vi "Logic.vi"(8 "error in (no error)":errorcluster, 11 "CIFPlugin in":refnum<class "CAN_Reader_CANsub_Plugin.lvclass">) -> (0 "error out":errorcluster, 3 "CIFPlugin out":refnum<class "CAN_Reader_CANsub_Plugin.lvclass">)   [LabVIEW 2021, in "CAN_Reader_CANsub_Plugin.lvclass"]
uses:
  CAN_Reader_CANsub_Plugin.lvclass
  CAN_Reader_CANsub_Plugin.lvclass/CAN_Reader_CANsub_Plugin.ctl
  Common/Typedef/Channels.ctl
  Common/CAN_Reader_CANsub_Common.lvlib
  <vilib>/CIF Foundation/CIF Core/CIFCore/Class/CIFCorePlugin.lvclass
  <vilib>/CIF Foundation/CIF Channels Core/ChannelCommon/typedef/TimeStamps.ctl
  <vilib>/CIF Foundation/CIF Channels Core/ChannelCommon/ChannelCommon.lvlib
  <vilib>/CIF Foundation/CIF Utilities/Time/Time_CIF_U.lvlib
  C:/Program Files/National Instruments/LabVIEW 2021/vi.lib/CIF Foundation/CIF Core/CIFCore/Class/CIFCorePlugin.lvclass
  <vilib>/CIF Foundation/CIF XNET CAN RW/XNET CAN RW.lvclass
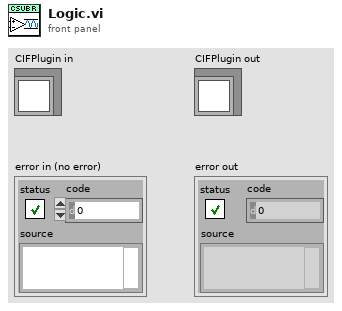
[diagram p1: front panel]
types:
  T1 = typedef "ChannelCommon.lvlib/TimeStamps.ctl" = cluster{"ClockID":u8, "T0":i64, "T_Out":i64}
  T2 = typedef "CAN_Reader_CANsub_Common.lvlib/Channels.ctl" = enum16{"CAN_Frames"}
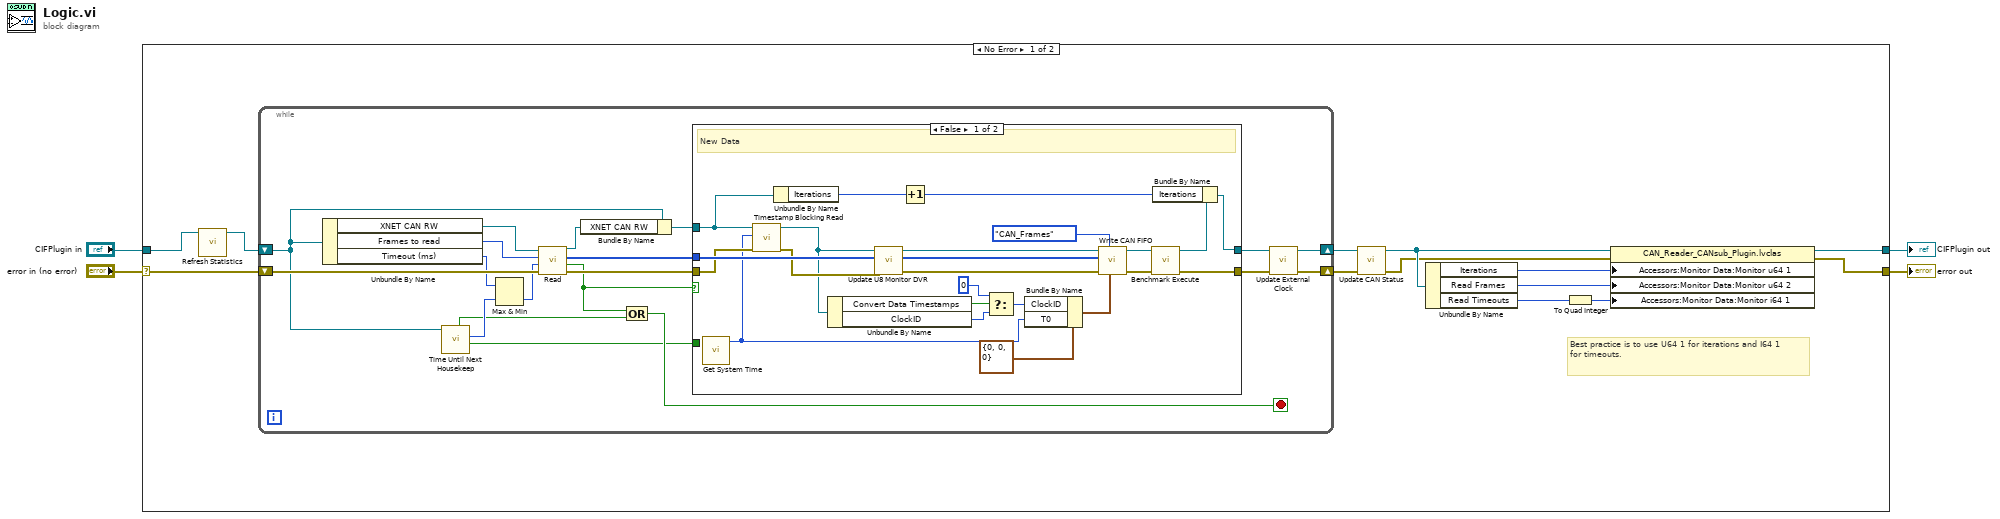
[diagram p0: block diagram]
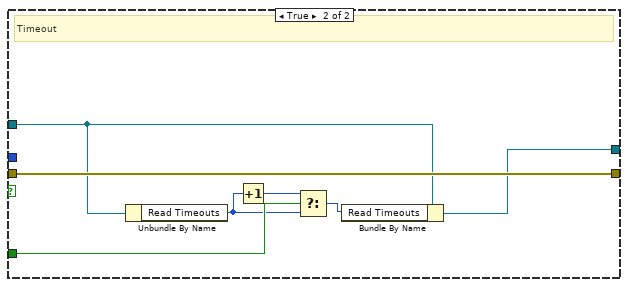
[diagram p2: hidden frame]
diagram:
  n1 = case shown="No Error" "error in (no error)" {
    selector: "error in (no error)" -> [w16 w68]
    tunnel: [w15 w68] -> w2
    tunnel: [w9 w67] -> w1
    tunnel: "CIFPlugin in" -> [w17 w67]
    frame No Error {
      # "Best practice is to use U64 1 for iterations and I64 1 for timeouts."
      n2 = call "Refresh Statistics.vi"("CIFPlugin in"=w17) -> ("CIFPlugin out"=w14:refnum<class "CAN_Reader_CANsub_Plugin.lvclass">)  [unwired: 10 in]
      n3 = while {
        shift-right: [w24] -> w7
        shift-left: w16 -> [w36]
        shift-right: [w25] -> w8
        shift-left: w14 -> [w31]
        stop <- w19 stop-if-true
        n4 = Unbundle By Name(w31) -> ("XNET CAN RW"=w35:refnum<class "XNET CAN RW.lvclass">, "Frames to read"=w34:i32, "Timeout (ms)"=w29:i32)
        n5 = call <vilib>:"Time Until Next Housekeep.vi"("CIFCorePlugin in"=w31) -> ("Timeout Valid"=w18:bool, "Time Until Next Housekeep (ms)"=w30:i32, "Housekeep Now"=w20:bool)  [unwired: 7 in, 1 out]
        n6 = Max & Min(x=w29, y=w30) -> (min(x,y)=w28:i32)  [unwired: 1 out]
        n7 = call-dynamic "Read.vi"("error in (no error)"=w36, "timeout (ms)"=w28, "number to read"=w34, "XNET_CAN_RW in"=w35) -> ("error out"=w22:errorcluster, "Timeout"=w21:bool, "pcap CAN Data"=w33:u8[], "XNET_CAN_RW out"=w32:refnum<class "XNET CAN RW.lvclass">)  [unwired: 3 in, 1 out]
        n8 = Bundle By Name(cluster=w31, "XNET CAN RW"=w32) -> (w23:refnum<class "CAN_Reader_CANsub_Plugin.lvclass">)
        n9 = Compound Arithmetic op=OR(w21, w20) -> (w19:bool)
        n10 = case shown="False" w21 {
          tunnel: w33 -> [w51 _]
          tunnel: w22 -> [w45 w66]
          tunnel: w23 -> [w42 w65]
          tunnel: [w38 w64] -> w27
          tunnel: [w46 w66] -> w26
          tunnel: w18 -> [_ w62]
          frame False {
            # "New Data"
            n11 = call <vilib>:"Get System Time.vi"() -> ("Time (ns)"=w37:i64)  [unwired: 5 in]
            n12 = call <vilib>:"Timestamp Blocking Read.vi"("error in (no error)"=w45, "RX Time"=w37, "CIFCorePlugin in"=w42) -> ("error out"=w44:errorcluster, "CIFCorePlugin out"=w43:refnum<class "CAN_Reader_CANsub_Plugin.lvclass">)  [unwired: 7 in]
            n13 = Unbundle By Name(w42) -> ("Iterations"=w41:u64)
            n14 = Unbundle By Name(w43) -> ("Convert Data Timestamps"=w57:bool, "ClockID"=w56:u8)
            n15 = call "Update U8 Monitor DVR.vi"("error in (no error)"=w44, "pcap CAN Data in"=w51, "CAN_Reader_NIXNET_Plugin in"=w43) -> ("error out"=w49:errorcluster, "pcap CAN Data out"=w50:u8[], "CAN_Reader_NIXNET_Plugin out"=w52:refnum<class "CAN_Reader_CANsub_Plugin.lvclass">)  [unwired: 6 in]
            n16 = Increment(x=w41) -> (x+1=w40:u64)
            n17 = Select(t=u8 0, s=w57, f=w56) -> (s? t:f=w54:u8)
            n18 = Bundle By Name(cluster=T1 {"ClockID"=0, "T0"=0, "T_Out"=0} ("FIFO Timestamps"), "ClockID"=w54, "T0"=w37) -> (w53:T1)
            n19 = call <vilib>:"Write CAN FIFO.vi"("FIFO Timestamps"=w53, "Channel Index"=Channels."CAN_Frames" ("Channels"), "error in (no error)"=w49, "Data"=w50, "CIFCorePlugin in"=w52) -> ("error out"=w47:errorcluster, "CIFCorePlugin out"=w48:refnum<class "CAN_Reader_CANsub_Plugin.lvclass">)  [unwired: 4 in, 1 out]
            n20 = call <vilib>:"Benchmark Execute.vi"("error in (no error)"=w47, "CIFCorePlugin in"=w48) -> ("error out"=w46:errorcluster, "CIFCorePlugin out"=w39:refnum<class "CAN_Reader_CANsub_Plugin.lvclass">)  [unwired: 8 in]
            n21 = Bundle By Name(cluster=w39, "Iterations"=w40) -> (w38:refnum<class "CAN_Reader_CANsub_Plugin.lvclass">)
          }
          frame True {
            # "Timeout"
            n22 = Unbundle By Name(w65) -> ("Read Timeouts"=w60:u64)
            n23 = Increment(x=w60) -> (x+1=w61:u64)
            n24 = Select(t=w61, s=w62, f=w60) -> (s? t:f=w63:u64)
            n25 = Bundle By Name(cluster=w65, "Read Timeouts"=w63) -> (w64:refnum<class "CAN_Reader_CANsub_Plugin.lvclass">)
          }
        }
        n26 = call "Update External Clock.vi"("error in (no error)"=w26, "CAN_Reader_NIXNET"=w27) -> ("error out"=w24:errorcluster, "CAN_Reader_NIXNET"=w25:refnum<class "CAN_Reader_CANsub_Plugin.lvclass">)  [unwired: 8 in]
      }
      n27 = call "Update CAN Status.vi"("error in (no error)"=w7, "CAN_Reader_NIXNET_Plugin"=w8) -> ("error out"=w5:errorcluster, "CAN_Reader_NIXNET_Plugin"=w6:refnum<class "CAN_Reader_CANsub_Plugin.lvclass">)  [unwired: 8 in]
      n28 = Unbundle By Name(w6) -> ("Iterations"=w10:u64, "Read Frames"=w11:u64, "Read Timeouts"=w13:u64)
      n29 = To Quad Integer(1:w13) -> (0:w12:i64)
      n30 = property class="CAN_Reader_CANsub_Plugin.lvclas"(reference=w6, error in=w5, "Accessors:Monitor Data:Monitor u64 1"=w10, "Accessors:Monitor Data:Monitor u64 2"=w11, "Accessors:Monitor Data:Monitor i64 1"=w12) -> (reference out=w9:refnum<class "CAN_Reader_CANsub_Plugin.lvclass">, error out=w15:errorcluster)
    }
    frame Error {
    }
  }
  "error out" <- w2
  "CIFPlugin out" <- w1
